vi "RemoteVI Complex Fixture Layout.vi"(0 "Panel":refnum<vi>, 1 "kind":string="layout", 2 "Host Panel":refnum<vi>, 11 "error in":errorcluster) -> (4 "layout":string, 5 "panes":string, 15 "error out":errorcluster)   [LabVIEW 2020]
doc: "Event-log helper of RemoteVI Complex Fixture.vi. Builds the layout lines of the log for every control RemoteVI Panel Controls.vi (RemoteVI.lvlib) finds on Panel - the top level of every pane, the selected page of a tab control and cluster elements, two levels deep -: kind TAB label TAB x y w h LF, the control's body in the coordinates of Host Panel's window: its Position and Bounds are converted from its pane's coordinates to panel coordinates ({LV.Pane} CvtPaneToPanelCoords on the pane of its top-level control; a cluster element's own OwningPane can name another pane), then to screen coordinates (CvtPanelToScreenCoords of Host Panel), minus the top-left of Host Panel's Front Panel Window:Panel Bounds - the same coordinates as RemoteVI's frame minus its origin message, for controls in every pane, on tab pages, in clusters and in a VI shown in a subpanel of Host Panel (whose pane coordinates convert into the host's panel). A visible label above the control is not part of the body (Position and Bounds include it). panes gets one line per pane of Panel: pane TAB index TAB x y w h LF, the visible part of the pane (its Position and Bounds as a GObject) in the same coordinates. Errors of the property reads go to error out."
uses:
  source/RemoteVI.lvlib
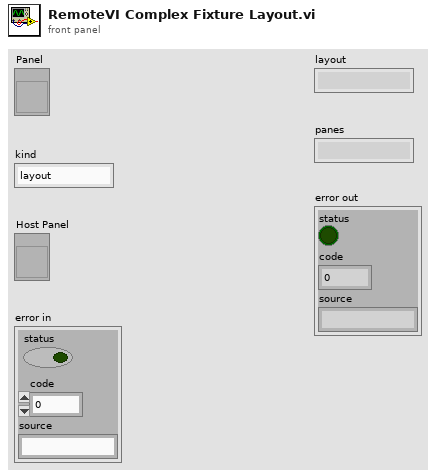
[diagram p1: front panel]
types:
  T1 = typedef "LVRectTypeDef.ctl" = cluster{"left":i16, "top":i16, "right":i16, "bottom":i16}
  T2 = typedef "LVPositionTypeDef.ctl" = cluster{"Left":i32, "Top":i32}
  T3 = typedef "LVBoundsTypeDef.ctl" = cluster{"Width":u32, "Height":u32}
  T4 = typedef "LVPointTypeDef.ctl" = cluster{"Horizontal":i16, "Vertical":i16}
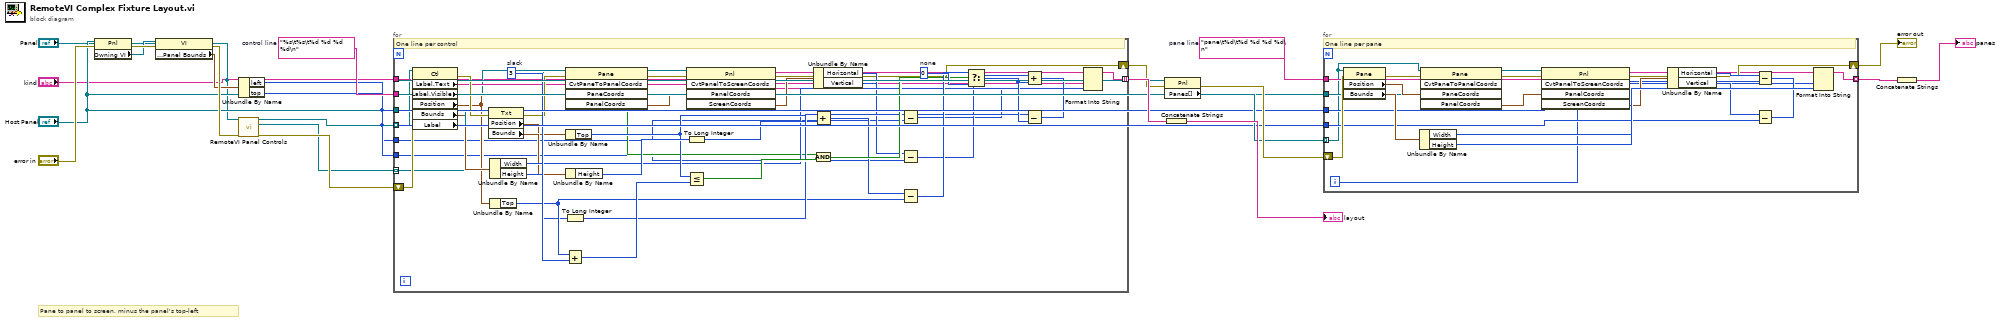
[diagram p0: block diagram]
diagram:
  w19 = "pane\t%d\t%d %d %d %d\n"  # pane line
  w14 = "%s\t%s\t%d %d %d %d\n"  # control line
  # "Pane to panel to screen, minus the panel's top-left"
  n1 = property class="Pnl"(reference="Host Panel", error in="error in") -> (error out=w6:errorcluster, "Owning VI"=w5:refnum<vi>)  [unwired: 1 out]
  n2 = property class="VI"(reference=w5, error in=w6) -> (error out=w8:errorcluster, "Front Panel Window:Panel Bounds"=w7:T1)  [unwired: 1 out]
  n3 = Unbundle By Name(w7) -> ("left"=w9:i16, "top"=w10:i16)
  n4 = call "RemoteVI Panel Controls.vi"("Panel"="Panel", "error in"=w8) -> ("Controls"=w11:refnum<vi>[], "Panes"=w12:refnum<vi>[], "error out"=w13:errorcluster)  [unwired: 11 in]
  n5 = for {
    tunnel: "kind" -> [w25]
    tunnel: w14 -> [w26]
    tunnel: "Host Panel" -> [w27]
    tunnel: w11 -> [w24] mode=indexing
    tunnel: w9 -> [w28]
    tunnel: w10 -> [w29]
    tunnel: w12 -> [w30] mode=indexing
    shift-right: [w32] -> w15
    shift-left: w13 -> [w31]
    tunnel: [w66] -> w16 mode=indexing
    w62 = 0  # none
    w57 = 3  # slack
    # "One line per control"
    n6 = property class="Ctl"(reference=w24, error in=w31) -> (error out=w38:errorcluster, "Label.Text"=w33:string, "Label.Visible"=w34:bool, "Position"=w35:T2, "Bounds"=w36:T3, "Label"=w37:refnum<vi>)  [unwired: 1 out]
    n7 = property class="Txt"(reference=w37, error in=w38) -> (error out=w41:errorcluster, "Position"=w39:T2, "Bounds"=w40:T3)  [unwired: 1 out]
    n8 = Unbundle By Name(w36) -> ("Width"=w49:u32, "Height"=w50:u32)
    n9 = Unbundle By Name(w35) -> ("Top"=w51:i32)
    n10 = Unbundle By Name(w39) -> ("Top"=w52:i32)
    n11 = Unbundle By Name(w40) -> ("Height"=w53:u32)
    n12 = To Long Integer(number=w50) -> (32bit integer=w55:i32)
    n13 = Add(x=w51, y=w57) -> (x+y=w58:i32)
    n14 = invoke class="Pane" method="CvtPaneToPanelCoords"(reference=w30, error in=w41, "PaneCoords"=w35) -> (error out=w42:errorcluster, "PanelCoords"=w43:T4)  [unwired: 2 in, 3 out]
    n15 = invoke class="Pnl" method="CvtPanelToScreenCoords"(reference=w27, error in=w42, "PanelCoords"=w43) -> (error out=w32:errorcluster, "ScreenCoords"=w44:T4)  [unwired: 2 in, 3 out]
    n16 = To Long Integer(number=w53) -> (32bit integer=w54:i32)
    n17 = Less Or Equal?(x=w52, y=w58) -> (x <= y?=w59:bool)
    n18 = Unbundle By Name(w44) -> ("Horizontal"=w45:i16, "Vertical"=w46:i16)
    n19 = Add(x=w52, y=w54) -> (x+y=w56:i32)
    n20 = And(x=w34, y=w59) -> (x .and. y?=w60:bool)
    n21 = Subtract(x=w45, y=w28) -> (x-y=w47:i16)
    n22 = Subtract(x=w46, y=w29) -> (x-y=w48:i16)
    n23 = Subtract(x=w56, y=w51) -> (x-y=w61:i32)
    n24 = Select(t=w61, s=w60, f=w62) -> (s? t:f=w63:i32)
    n25 = Add(x=w48, y=w63) -> (x+y=w64:i32)
    n26 = Subtract(x=w55, y=w63) -> (x-y=w65:i32)
    n27 = Format Into String(format string=w26, w25, w33, w47, w64, w49, w65) -> (resulting string=w66:string)  [unwired: 2 in, 1 out]
  }
  n28 = property class="Pnl"(reference="Panel", error in=w15) -> (error out=w18:errorcluster, "Panes[]"=w17:refnum<vi>[])  [unwired: 1 out]
  n29 = Concatenate Strings(w16) -> (→"layout":string)
  n30 = for {
    tunnel: w19 -> [w69]
    tunnel: "Host Panel" -> [w70]
    tunnel: w9 -> [w71]
    tunnel: w10 -> [w72]
    tunnel: w17 -> [w68] mode=indexing
    shift-right: [w74] -> w20
    shift-left: w18 -> [w73]
    tunnel: [w87] -> w21 mode=indexing
    i -> [w67]
    # "One line per pane"
    n31 = property class="Pane"(reference=w68, error in=w73) -> (error out=w77:errorcluster, "Position"=w75:T2, "Bounds"=w76:T3)  [unwired: 1 out]
    n32 = Unbundle By Name(w76) -> ("Width"=w85:u32, "Height"=w86:u32)
    n33 = invoke class="Pane" method="CvtPaneToPanelCoords"(reference=w68, error in=w77, "PaneCoords"=w75) -> (error out=w78:errorcluster, "PanelCoords"=w79:T4)  [unwired: 2 in, 3 out]
    n34 = invoke class="Pnl" method="CvtPanelToScreenCoords"(reference=w70, error in=w78, "PanelCoords"=w79) -> (error out=w74:errorcluster, "ScreenCoords"=w80:T4)  [unwired: 2 in, 3 out]
    n35 = Unbundle By Name(w80) -> ("Horizontal"=w81:i16, "Vertical"=w82:i16)
    n36 = Subtract(x=w81, y=w71) -> (x-y=w83:i16)
    n37 = Subtract(x=w82, y=w72) -> (x-y=w84:i16)
    n38 = Format Into String(format string=w69, w67, w83, w84, w85, w86) -> (resulting string=w87:string)  [unwired: 2 in, 1 out]
  }
  "error out" <- w20
  n39 = Concatenate Strings(w21) -> (→"panes":string)
